vi "2.1.vi"() -> ()   [LabVIEW 2013]
panel:
  out "Кількість ітерацій":dbl format="%#.6g"
  out "Поточне випадкове число":dbl format="%#.6g"
  in  "Задане число для порівняння":dbl=50.0 min=0.0 max=10000.0 step=1.0
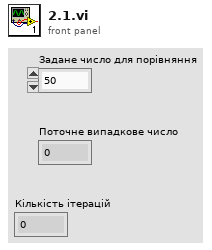
[diagram p1: front panel]
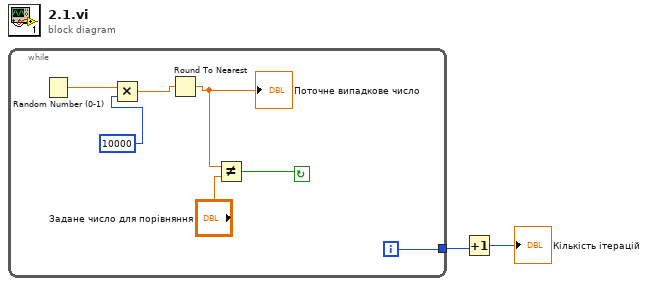
[diagram p0: block diagram]
diagram:
  n1 = while {
    tunnel: [w4] -> w2
    i -> [w4]
    stop <- w5 continue-if-true
    n2 = Random Number (0-1)() -> (number: 0 to 1=w3:dbl)
    n3 = Multiply(x=w3, y=10000) -> (x*y=w8:dbl)
    n4 = Round To Nearest(number=w8) -> (nearest integer value=w6:dbl)
    "Поточне випадкове число" <- w6
    n5 = Not Equal?(x=w6, y="Задане число для порівняння") -> (x != y?=w5:bool)
  }
  n6 = Increment(x=w2) -> (x+1=→"Кількість ітерацій":i32)
